vi "Show.vi"(8 "error in (no error)":errorcluster, 11 "ToastBuilder in":refnum<class "ToastBuilder.lvclass">) -> (0 "error out":errorcluster, 3 "ToastBuilder out":refnum<class "ToastBuilder.lvclass">)   [LabVIEW 2026, in "ToastNotification.lvlib" / "ToastBuilder.lvclass"]
doc: "ToastSource display override for ToastBuilder. Display the composed toast through the native toolkit. Skipped on incoming error; return the same builder without closing it. ToastService.Show delegates here through ToastSource. Register the service handler before display if activation replies are required. The caller retains ownership."
uses:
  ToastBuilder.lvclass
  ToastBuilder.lvclass/ToastBuilder.ctl
  Read Builder Reference.vi
  Write Builder Reference.vi
  Toast Native/Toast Native.lvlib
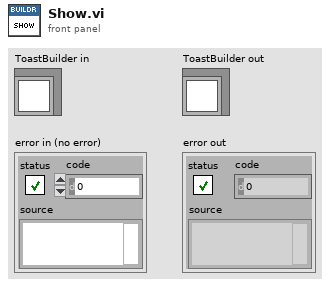
[diagram p1: front panel]
types:
  T1 = typedef "ToastNotification.lvlib/ToastBuilder.lvclass/Builder Reference.ctl" = refnum<k24>
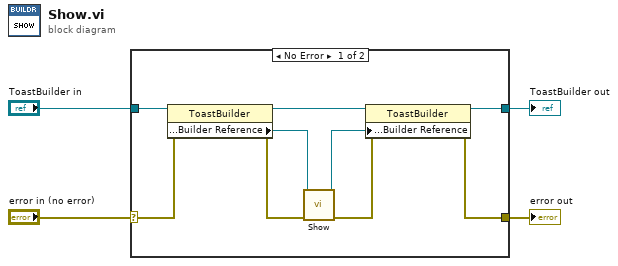
[diagram p0: block diagram]
diagram:
  n1 = case shown="No Error" "error in (no error)" {
    selector: "error in (no error)" -> [w10 w15]
    tunnel: [w9 w15] -> w3
    tunnel: [w11 w14] -> w1
    tunnel: "ToastBuilder in" -> [w13 w14]
    frame No Error {
      n2 = property class="ToastBuilder"(reference=w13, error in=w10) -> (reference out=w12:refnum<class "ToastBuilder.lvclass">, error out=w8:errorcluster, "Public:Properties:Builder Reference"=w6:T1)
      n3 = call "Show.vi"("error in (no error)"=w8, "reference"=w6) -> ("error out"=w7:errorcluster, "reference out"=w5:refnum<k24>)  [unwired: 8 in]
      n4 = property class="ToastBuilder"(reference=w12, error in=w7, "Public:Properties:Builder Reference"=w5) -> (reference out=w11:refnum<class "ToastBuilder.lvclass">, error out=w9:errorcluster)
    }
    frame Error {
    }
  }
  "error out" <- w3
  "ToastBuilder out" <- w1
